vi "ClassList Playground.vi"() -> ()   [LabVIEW 2019]
uses:
  Classes/Subpanel/Edit/Edit/Edit.lvclass
  Classes/Settings/Setting Database/Setting Database.lvclass
  C:/Program Files (x86)/National Instruments/LabVIEW 2019/vi.lib/JKI/JKI SMO/SMO/SMO.lvclass
  Classes/Settings/Setting Database/Typedefs/PrivateEvents--Setting Database.Refresh.ctl
  Classes/Settings/Setting Database/Typedefs/PrivateEvents--Setting Database.SetActivePath.ctl
  Classes/Settings/Setting Database/Typedefs/PrivateEvents--Setting Database.Add To Group.ctl
  Classes/Settings/Setting Database/Typedefs/PrivateEvents--Setting Database.SetActiveRectangle.ctl
  Classes/Subpanel/Manager/Subpanel.Edit.lvclass
  C:/Users/Albro/Documents/GitHub/AFM-Lithography/lvsrc/Classes/Subpanel/Subpanel.lvclass
  Classes/Subpanel/Edit/Edit.Path/Edit.Path.lvclass
  <vilib>/JKI/JKI SMO/SMO/SMO.lvclass
  Classes/Subpanel/Subpanel.lvclass
  C:/Users/Albro/Documents/GitHub/AFM-Lithography/lvsrc/Classes/Subpanel/Edit/Edit/Edit.lvclass
panel:
  out "Array":T1(array[cluster])
  in  "Key":string="p"
  out "key not found?":bool
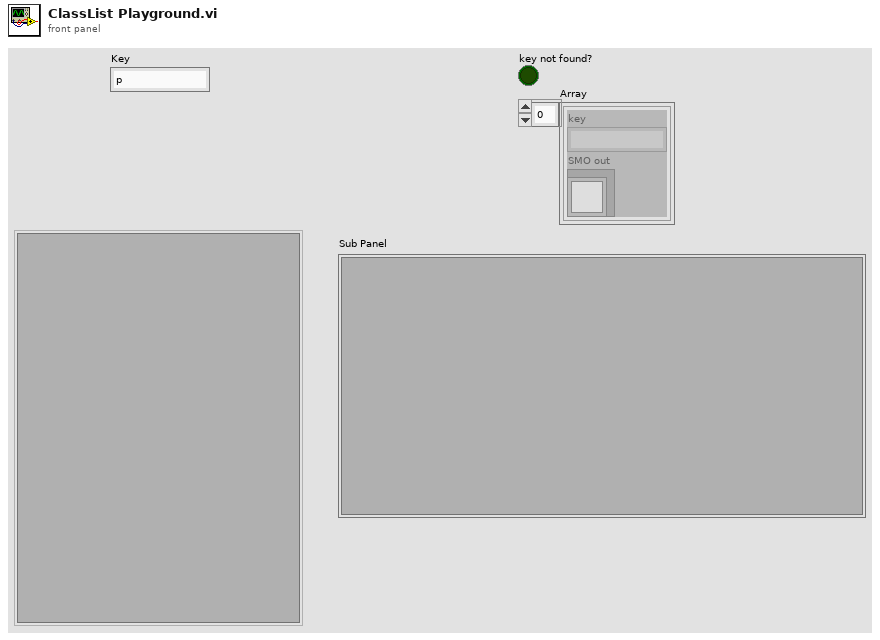
[diagram p1: front panel]
types:
  T1 = cluster{"key":string, "SMO out":refnum<class "Edit.lvclass">}[]
  T2 = typedef "Setting Database.lvclass/PrivateEvents--Setting Database.SetActiveRectangle.ctl" = string
  T3 = typedef "Setting Database.lvclass/PrivateEvents--Setting Database.Add To Group.ctl" = cluster{"Name":string, "Group":string}
  T4 = typedef "Setting Database.lvclass/PrivateEvents--Setting Database.SetActivePath.ctl" = string
  T5 = typedef "Setting Database.lvclass/PrivateEvents--Setting Database.Refresh.ctl" = cluster{"Paths":string[], "Rectangles":string[], "Funnels":string[], "Dots":string[]}
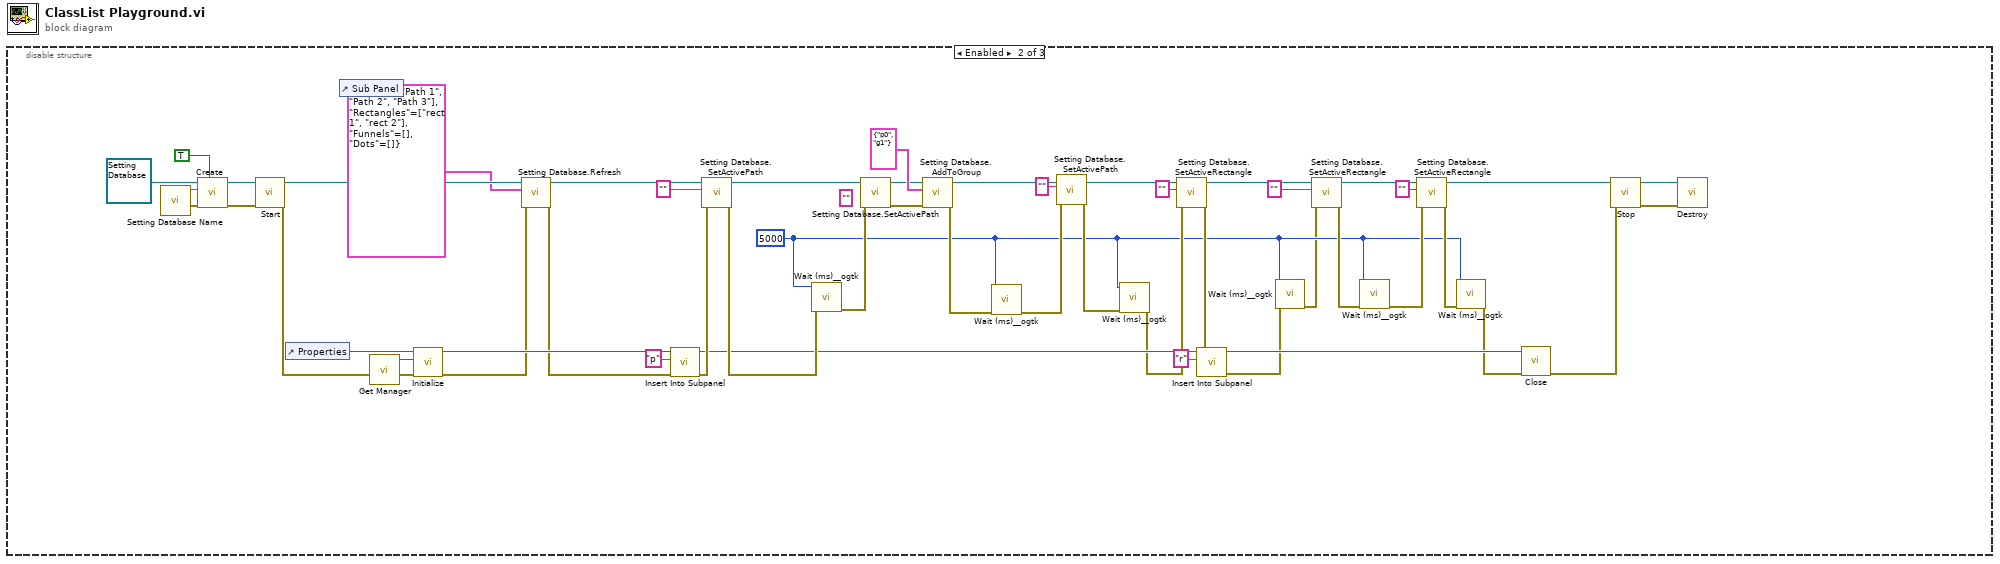
[diagram p0: block diagram]
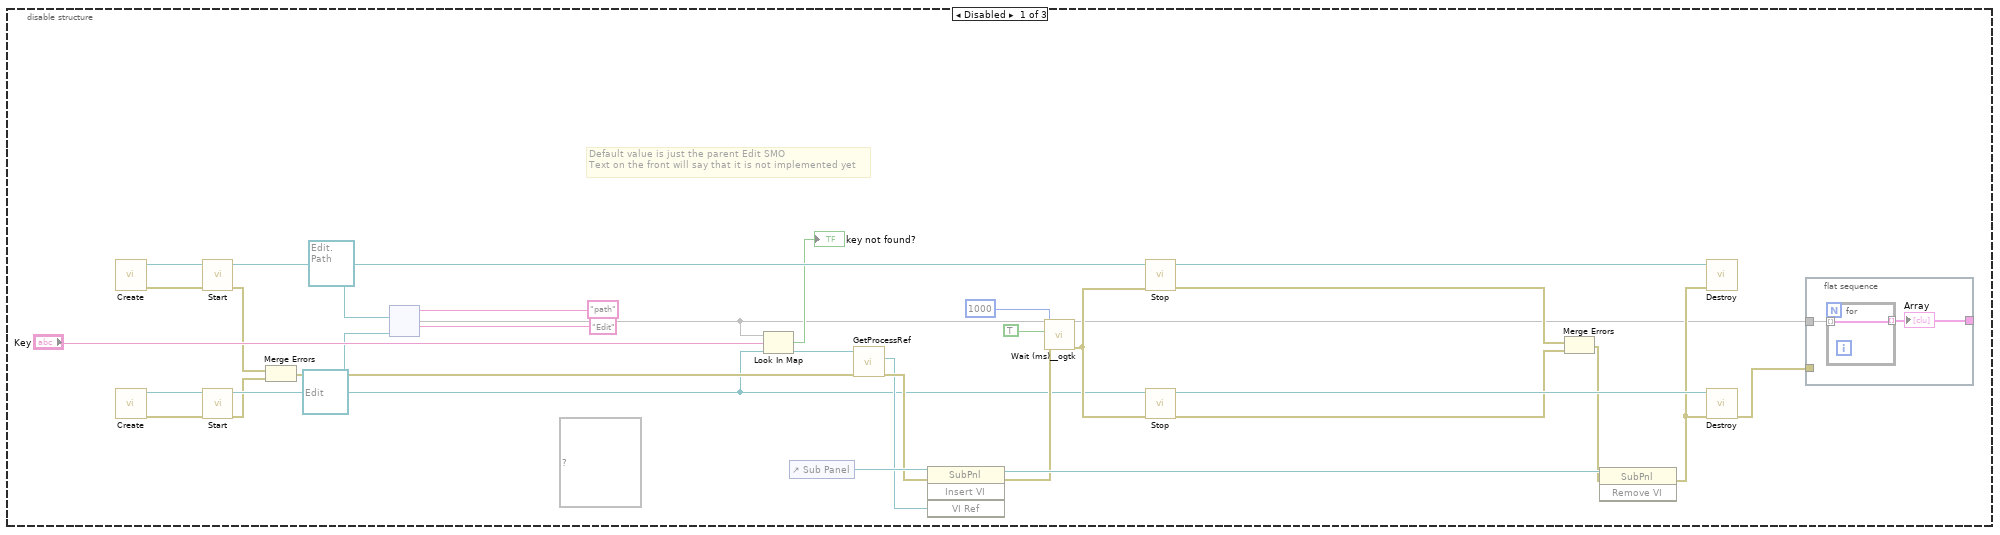
[diagram p2: hidden frame]
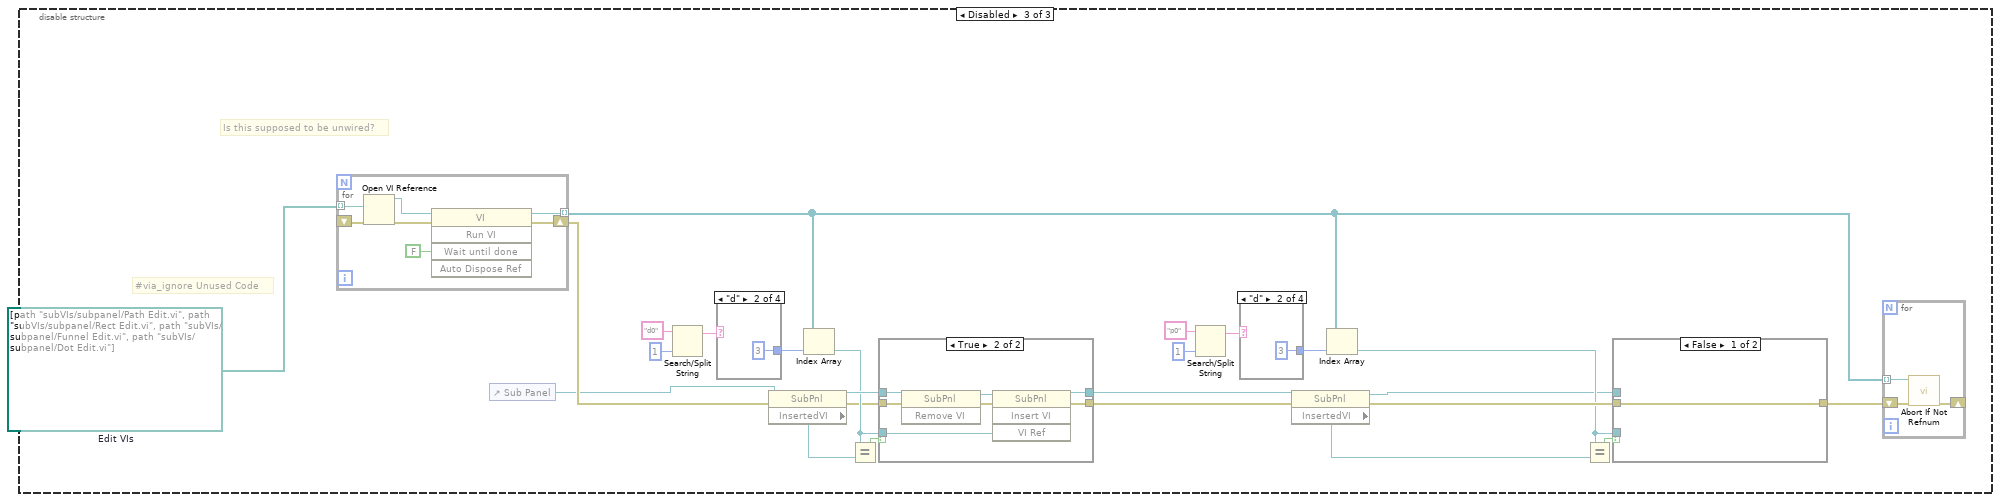
[diagram p3: hidden frame]
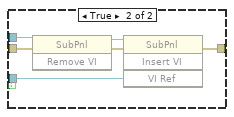
[diagram p4: hidden frame]
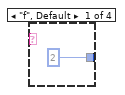
[diagram p5: hidden frame]
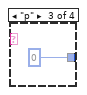
[diagram p6: hidden frame]
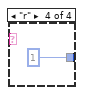
[diagram p7: hidden frame]
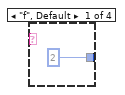
[diagram p9: hidden frame]
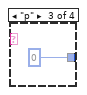
[diagram p10: hidden frame]
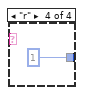
[diagram p11: hidden frame]
diagram:
  n1 = disable-structure shown="Enabled" {
    frame Disabled {
      (unwired) map{string, refnum<class "Edit.lvclass">} {} ("map")
      # "Default value is just the parent Edit SMO\nText on the front will say that it is not implemented yet"
      n2 = call <vilib>:"Create.vi"("SMO"=refnum<class "Edit.Path.lvclass"> refnum ("Edit.Path.lvclass")) -> ("error out"=w16:errorcluster, "SMO out"=w29:refnum<class "Edit.Path.lvclass">)  [unwired: 8 in, 1 out]
      n3 = call <vilib>:"Create.vi"("SMO"=refnum<class "Edit.lvclass"> refnum ("Edit.lvclass")) -> ("error out"=w12:errorcluster, "SMO out"=w30:refnum<class "Edit.lvclass">)  [unwired: 8 in, 1 out]
      n4 = call <vilib>:"Start.vi"("error in (no error)"=w16, "SMO"=w29) -> ("error out"=w15:errorcluster, "SMO out"=w24:refnum<class "Edit.Path.lvclass">)  [unwired: 8 in]
      n5 = call <vilib>:"Start.vi"("error in (no error)"=w12, "SMO"=w30) -> ("error out"=w14:errorcluster, "SMO out"=w3:refnum<class "Edit.lvclass">)  [unwired: 8 in]
      n6 = Merge Errors(w15, w14) -> (w13:errorcluster)
      n7 = node("path" ("key"), w24, "Edit" ("key"), w3) -> (w1:map{string, refnum<class "Edit.lvclass">})
      n8 = Look In Map(map=w1, key="Key", default value=w3) -> (key not found?=→"key not found?":bool, value=w26:refnum<class "Edit.lvclass">)
      n9 = control-ref of="Sub Panel"() -> (w10:refnum<vi>)
      n10 = call "GetProcessRef.vi"("error in (no error)"=w13, "Edit in"=w26) -> ("error out"=w6:errorcluster, "Static VI Ref"=w5:refnum<vi>)  [unwired: 7 in, 1 out]
      n11 = invoke class="SubPnl" method="Insert VI"(reference=w10, error in=w6, "VI Ref"=w5) -> (reference out=w23:refnum<vi>, error out=w7:errorcluster)  [unwired: 1 in, 2 out]
      n12 = call <userlib>:"Wait (ms)__ogtk.vi"("error in (no error)"=w7, "Wait on Error (FALSE)"=TRUE, "milliseconds to wait"=u32 1000) -> ("error out"=w25:errorcluster)  [unwired: 7 in, 1 out]
      n13 = call <vilib>:"Stop.vi"("error in (no error)"=w25, "SMO"=w24) -> ("error out"=w8:errorcluster, "SMO out"=w21:refnum<class "Edit.Path.lvclass">)  [unwired: 8 in]
      n14 = call <vilib>:"Stop.vi"("error in (no error)"=w25, "SMO"=w3) -> ("error out"=w18:errorcluster, "SMO out"=w22:refnum<class "Edit.lvclass">)  [unwired: 8 in]
      n15 = Merge Errors(w8, w18) -> (w19:errorcluster)
      n16 = invoke class="SubPnl" method="Remove VI"(reference=w23, error in=w19) -> (error out=w17:errorcluster)  [unwired: 1 in, 2 out]
      n17 = call <vilib>:"Destroy.vi"("error in (no error)"=w17, "SMO"=w21) -> ()  [unwired: 9 in, 1 out]
      n18 = call <vilib>:"Destroy.vi"("error in (no error)"=w17, "SMO"=w22) -> ("error out"=w2:errorcluster)  [unwired: 9 in]
      n19 = flat-sequence {
        tunnel: w1 -> [w34]
        tunnel: w2 -> [_]
        tunnel: [w33] -> _
        frame #0 {
          n20 = for {
            tunnel: w34 -> [w35] mode=indexing
            tunnel: [w35] -> w33 mode=indexing
          }
          "Array" <- w33
        }
      }
    }
    frame Enabled {
      (unwired) T4 "" ("SetActivePath")
      w42 = u32 5000 ("milliseconds to wait")
      n21 = call "Setting Database Name.vi"() -> ("error out"=w76:errorcluster, "Name"=w77:string)  [unwired: 10 in]
      n22 = call <vilib>:"Create.vi"("Shared Resource (F)"=TRUE, "error in (no error)"=w76, "Subsystem Name (optional)"=w77, "SMO"=refnum<class "Setting Database.lvclass"> refnum ("Setting Database.lvclass")) -> ("error out"=w80:errorcluster, "SMO out"=w81:refnum<class "Setting Database.lvclass">)  [unwired: 5 in, 1 out]
      n23 = call <vilib>:"Start.vi"("error in (no error)"=w80, "SMO"=w81) -> ("error out"=w75:errorcluster, "SMO out"=w71:refnum<class "Setting Database.lvclass">)  [unwired: 8 in]
      n24 = control-ref of="Properties"() -> (w72:refnum<vi>)
      n25 = control-ref of="Sub Panel"() -> ()  [unwired: 1 out]
      n26 = call "Get Manager.vi"("error in (no error)"=w75) -> ("error out"=w74:errorcluster, "Subpanel.Edit"=w73:refnum<class "Subpanel.Edit.lvclass">)  [unwired: 9 in]
      n27 = call "Initialize.vi"("error in (no error)"=w74, "Subpanel.lvclass"=w73, "Sub Panel"=w72) -> ("error out"=w61:errorcluster, "Subpanel out"=w86:refnum<class "Subpanel.Edit.lvclass">)  [unwired: 7 in]
      n28 = call "Setting Database.Refresh.vi"("error in (no error)"=w61, "Initialize"=T5 {"Paths"=["Path 1", "Path 2", "Path 3"], "Rectangles"=["rect 1", "rect 2"], "Funnels"=[], "Dots"=[]}, "Setting Database"=w71) -> ("error out"=w60:errorcluster, "Setting Database out"=w68:refnum<class "Setting Database.lvclass">)  [unwired: 7 in]
      n29 = call "Insert Into Subpanel.vi"("error in (no error)"=w60, "Key"="p", "Subpanel.lvclass"=w86) -> ("error out"=w59:errorcluster, "Subpanel out"=w53:refnum<class "Subpanel.Edit.lvclass">)  [unwired: 7 in]
      n30 = call "Setting Database.SetActivePath.vi"("error in (no error)"=w59, "SetActivePath"=T4 "", "Setting Database"=w68) -> ("error out"=w65:errorcluster, "Setting Database out"=w67:refnum<class "Setting Database.lvclass">)  [unwired: 7 in]
      n31 = call <userlib>:"Wait (ms)__ogtk.vi"("error in (no error)"=w65, "milliseconds to wait"=w42) -> ("error out"=w64:errorcluster)  [unwired: 8 in, 1 out]
      n32 = call "Setting Database.SetActivePath.vi"("error in (no error)"=w64, "Setting Database"=w67) -> ("error out"=w56:errorcluster, "Setting Database out"=w57:refnum<class "Setting Database.lvclass">)  [unwired: 8 in]
      n33 = call "Setting Database.AddToGroup.vi"("error in (no error)"=w56, "Add To Group"=T3 {"Name"="p0", "Group"="g1"}, "Setting Database"=w57) -> ("error out"=w55:errorcluster, "Setting Database out"=w51:refnum<class "Setting Database.lvclass">)  [unwired: 7 in]
      n34 = call <userlib>:"Wait (ms)__ogtk.vi"("error in (no error)"=w55, "milliseconds to wait"=w42) -> ("error out"=w62:errorcluster)  [unwired: 8 in, 1 out]
      n35 = call "Setting Database.SetActivePath.vi"("error in (no error)"=w62, "SetActivePath"=T4 "", "Setting Database"=w51) -> ("error out"=w63:errorcluster)  [unwired: 7 in, 1 out]
      n36 = call <userlib>:"Wait (ms)__ogtk.vi"("error in (no error)"=w63, "milliseconds to wait"=w42) -> ("error out"=w48:errorcluster)  [unwired: 8 in, 1 out]
      n37 = call "Setting Database.SetActiveRectangle.vi"("error in (no error)"=w48, "SetActiveRectangle"=T2 "", "Setting Database"=w51) -> ("error out"=w47:errorcluster, "Setting Database out"=w40:refnum<class "Setting Database.lvclass">)  [unwired: 7 in]
      n38 = call "Insert Into Subpanel.vi"("error in (no error)"=w47, "Key"="r", "Subpanel.lvclass"=w53) -> ("error out"=w49:errorcluster, "Subpanel out"=w52:refnum<class "Subpanel.Edit.lvclass">)  [unwired: 7 in]
      n39 = call <userlib>:"Wait (ms)__ogtk.vi"("error in (no error)"=w49, "milliseconds to wait"=w42) -> ("error out"=w38:errorcluster)  [unwired: 8 in, 1 out]
      n40 = call "Setting Database.SetActiveRectangle.vi"("error in (no error)"=w38, "SetActiveRectangle"=T2 "", "Setting Database"=w40) -> ("error out"=w46:errorcluster, "Setting Database out"=w41:refnum<class "Setting Database.lvclass">)  [unwired: 7 in]
      n41 = call <userlib>:"Wait (ms)__ogtk.vi"("error in (no error)"=w46, "milliseconds to wait"=w42) -> ("error out"=w44:errorcluster)  [unwired: 8 in, 1 out]
      n42 = call "Setting Database.SetActiveRectangle.vi"("error in (no error)"=w44, "SetActiveRectangle"=T2 "", "Setting Database"=w41) -> ("error out"=w43:errorcluster, "Setting Database out"=w39:refnum<class "Setting Database.lvclass">)  [unwired: 7 in]
      n43 = call <userlib>:"Wait (ms)__ogtk.vi"("error in (no error)"=w43, "milliseconds to wait"=w42) -> ("error out"=w37:errorcluster)  [unwired: 8 in, 1 out]
      n44 = call "Close.vi"("error in (no error)"=w37, "Subpanel.lvclass"=w52) -> ("error out"=w84:errorcluster)  [unwired: 8 in, 1 out]
      n45 = call <vilib>:"Stop.vi"("error in (no error)"=w84, "SMO"=w39) -> ("error out"=w83:errorcluster, "SMO out"=w82:refnum<class "Setting Database.lvclass">)  [unwired: 8 in]
      n46 = call <vilib>:"Destroy.vi"("error in (no error)"=w83, "SMO"=w82) -> ()  [unwired: 9 in, 1 out]
    }
    frame Disabled {
      w111 = path[] [path "subVIs/subpanel/Path Edit.vi", path "subVIs/subpanel/Rect Edit.vi", path "subVIs/subpanel/Funnel Edit.vi", path "subVIs/subpanel/Dot Edit.vi"]  # Edit VIs
      # "#via_ignore Unused Code"
      # "Is this supposed to be unwired?"
      n47 = for {
        tunnel: [w140] -> w87 mode=indexing
        shift-right: [w143] -> w106
        shift-left: _ -> [w144]
        tunnel: w111 -> [w139] mode=indexing
        # "Load and run Plugin VIs"
        n48 = Open VI Reference(vi path=w139, error in (no error)=w144) -> (vi reference=w141:refnum<vi>, error out=w145:errorcluster)  [unwired: 4 in]
        n49 = invoke on="Invoke Node" class="VI" method="Run VI"(reference=w141, error in=w145, "Wait until done"=FALSE ("Wait Until Done")) -> (reference out=w140:refnum<vi>, error out=w143:errorcluster)  [unwired: 2 in, 3 out]
      }
      n50 = control-ref of="Sub Panel"() -> (w100:refnum<vi>)
      n51 = Search/Split String(string="d0", offset (0)=1) -> (substring before match=w109:string)  [unwired: 1 in, 2 out]
      n52 = case shown="\"d\"" w109 {
        tunnel: [2 3 0 1] -> w110
        frame "f", Default {
        }
        frame "d" {
        }
        frame "p" {
        }
        frame "r" {
        }
      }
      n53 = property class="SubPnl"(reference=w100, error in=w106) -> (reference out=w104:refnum<vi>, error out=w102:errorcluster, "InsertedVI"=w107:refnum<vi>)
      n54 = Index Array(array=w87, index=w110) -> (element=w103:refnum<vi>)
      n55 = Equal?(x=w103, y=w107) -> (x = y?=w105:bool)
      n56 = case shown="True" w105 {
        tunnel: w104 -> [w126 w132]
        tunnel: w103 -> [_ w131]
        tunnel: w102 -> [w127 w130]
        tunnel: [w127 w129] -> w90
        tunnel: [w126 w128] -> w89
        frame False {
        }
        frame True {
          n57 = invoke on="Invoke Node" class="SubPnl" method="Remove VI"(reference=w132, error in=w130) -> (reference out=w133:refnum<vi>, error out=w134:errorcluster)  [unwired: 1 in, 1 out]
          n58 = invoke on="Invoke Node" class="SubPnl" method="Insert VI"(reference=w133, error in=w134, "VI Ref"=w131) -> (reference out=w128:refnum<vi>, error out=w129:errorcluster)  [unwired: 1 in, 2 out]
        }
      }
      n59 = Search/Split String(string="p0", offset (0)=1) -> (substring before match=w92:string)  [unwired: 1 in, 2 out]
      n60 = case shown="\"d\"" w92 {
        tunnel: [2 3 0 1] -> w91
        frame "f", Default {
        }
        frame "d" {
        }
        frame "p" {
        }
        frame "r" {
        }
      }
      n61 = property class="SubPnl"(reference=w89, error in=w90) -> (reference out=w96:refnum<vi>, error out=w98:errorcluster, "InsertedVI"=w94:refnum<vi>)
      n62 = Index Array(array=w87, index=w91) -> (element=w97:refnum<vi>)
      n63 = Equal?(x=w97, y=w94) -> (x = y?=w95:bool)
      n64 = case shown="False" w95 {
        tunnel: w96 -> [_ w119]
        tunnel: w97 -> [_ w118]
        tunnel: w98 -> [w115 w117]
        tunnel: [w115 w116] -> w88
        frame False {
        }
        frame True {
          n65 = invoke on="Invoke Node" class="SubPnl" method="Remove VI"(reference=w119, error in=w117) -> (reference out=w120:refnum<vi>, error out=w121:errorcluster)  [unwired: 1 in, 1 out]
          n66 = invoke on="Invoke Node" class="SubPnl" method="Insert VI"(reference=w120, error in=w121, "VI Ref"=w118) -> (error out=w116:errorcluster)  [unwired: 1 in, 3 out]
        }
      }
      n67 = for {
        tunnel: w87 -> [w112] mode=indexing
        shift-right: [w113] -> _
        shift-left: w88 -> [w114]
        n68 = call "Abort If Not Refnum.vi"("error in (no error)"=w114, "VI in"=w112) -> ("error out"=w113:errorcluster)  [unwired: 9 in]
      }
    }
  }
